vi "Start Record.vi"(8 "error in (no error)":errorcluster, 10 "tdms ref":refnum<k34>, 11 "DMM Engine":refnum<class "DMM Engine.lvclass">) -> (0 "error out":errorcluster, 3 "DMM Engine out":refnum<class "DMM Engine.lvclass">)   [LabVIEW 2025, in "DMM.lvlib" / "DMM Engine.lvclass"]
uses:
  DMM Engine.lvclass
  DMM Engine.lvclass/DMM Engine.ctl
  DMM configuration/DMM configuration.lvclass
  DMM Channel/DMM Channel.lvclass
  Users/Public/Documents/Sandia National Labs/TSS Plugin/Abstract.lvlibp/Channel configuration/Channel configuration.lvclass
  DMM Instrument/DMM Instrument.lvclass
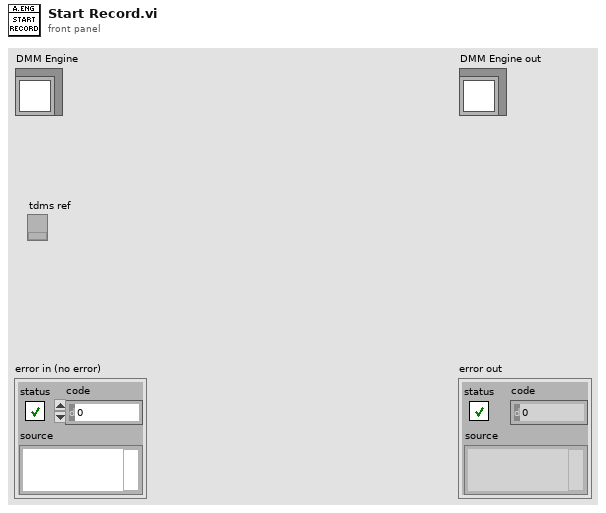
[diagram p1: front panel]
types:
  T1 = typedef "Abstract.lvlibp/Abstract Engine.lvclass/Engine Cluster.ctl" = cluster{"Initialized":bool, "IP Address":string, "Engine Type":string, "InstrumentMap":map{string, cluster{"Initialized":bool, "IP Address":string, "Instr Type":string, "Channels":cluster{"Enable":bool, "Alias":string}[]}}}
  T2 = typedef "Abstract.lvlibp/Instrument configuration.lvclass/Default Instrument.ctl" = cluster{"InstType":string, "Address":string, "SW Alias":string, "Description":string, "Enabled":bool}
  T3 = typedef "Abstract.lvlibp/Channel configuration.lvclass/Default Channel.ctl" = cluster{"SW Alias":string, "Enabled":bool, "Class":string, "Type":T4, "AI Parameter":cluster{"Upper limit":dbl, "Lower limit":dbl, "Unit":T4}}
  T4 = typedef "Abstract.lvlibp/Channel configuration.lvclass/Data Type.ctl" = string
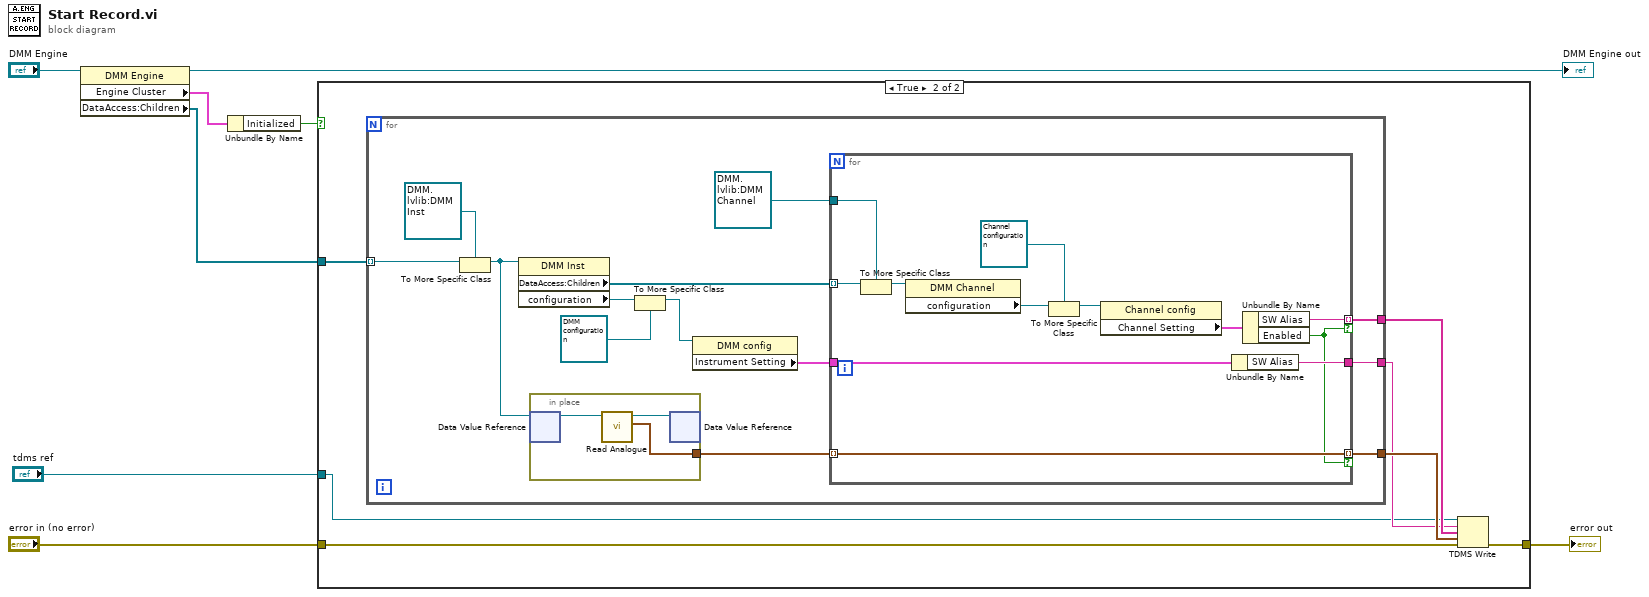
[diagram p0: block diagram]
diagram:
  n1 = property class="DMM Engine"(reference="DMM Engine") -> (reference out=→"DMM Engine out":refnum<class "DMM Engine.lvclass">, "Engine Cluster"=w5:T1, "DataAccess:Children"=w1:refnum<data-value>[])  [unwired: 1 in, 1 out]
  n2 = Unbundle By Name(w5) -> ("Initialized"=w8:bool)
  n3 = case shown="True" w8 {
    tunnel: "error in (no error)" -> [w9 w11]
    tunnel: [w9 w15] -> w6
    tunnel: "tdms ref" -> [_ w10]
    tunnel: w1 -> [_ w16]
    frame False {
    }
    frame True {
      n4 = for {
        tunnel: w16 -> [w26] mode=indexing
        tunnel: [w29] -> w14
        tunnel: [w28] -> w13
        tunnel: [w27] -> w12
        n5 = To More Specific Class(target class=refnum<data-value> refnum ("data value reference"), reference=w26) -> (specific class reference=w19:refnum<data-value>)  [unwired: 1 in, 1 out]
        n6 = property class="DMM Inst"(reference=w19) -> ("DataAccess:Children"=w20:refnum<data-value>[], "configuration"=w22:refnum<class "CEF_serializable configuration.lvclass">)  [unwired: 1 in, 2 out]
        n7 = in-place {
          in-place-border: [w30] -> w18
          n8 = in-place-dvr #1(w19) -> (w32:refnum<class "DMM Instrument.lvclass">)  [unwired: 1 out]
          n9 = call-dynamic "Read Analogue.vi"("Abstract DMM in"=w32) -> ("Waveforms"=w30:waveform(dbl)[], "Abstract DMM out"=w31:refnum<class "DMM Instrument.lvclass">)  [unwired: 8 in, 1 out]
          n10 = in-place-dvr #1(w31) -> ()  [unwired: 2 out]
        }
        n11 = To More Specific Class(target class=refnum<class "DMM configuration.lvclass"> refnum ("DMM.lvlib:DMM config"), reference=w22) -> (specific class reference=w24:refnum<class "DMM configuration.lvclass">)  [unwired: 1 in, 1 out]
        n12 = property class="DMM config"(reference=w24) -> ("Instrument Setting"=w21:T2)  [unwired: 1 in, 2 out]
        n13 = for {
          tunnel: w21 -> [w43]
          tunnel: w18 -> [w37] mode=indexing
          tunnel: [w37] -> w29 mode=indexing if=w35
          tunnel: [w38] -> w28 mode=indexing if=w35
          tunnel: [w36] -> w27
          tunnel: w20 -> [w34] mode=indexing
          tunnel: refnum<data-value> refnum ("data value reference") -> [w33]
          n14 = To More Specific Class(target class=w33, reference=w34) -> (specific class reference=w44:refnum<data-value>)  [unwired: 1 in, 1 out]
          n15 = property class="DMM Channel"(reference=w44) -> ("configuration"=w42:refnum<class "CEF_serializable configuration.lvclass">)  [unwired: 1 in, 2 out]
          n16 = To More Specific Class(target class=refnum<class "Channel configuration.lvclass"> refnum ("Abstract.lvlibp:Channel config"), reference=w42) -> (specific class reference=w40:refnum<class "Channel configuration.lvclass">)  [unwired: 1 in, 1 out]
          n17 = property class="Channel config"(reference=w40) -> ("Channel Setting"=w39:T3)  [unwired: 1 in, 2 out]
          n18 = Unbundle By Name(w43) -> ("SW Alias"=w36:string)
          n19 = Unbundle By Name(w39) -> ("SW Alias"=w38:string, "Enabled"=w35:bool)
        }
      }
      n20 = TDMS Write(0:w10, 5:w12, 7:w13, 9:w14, 11:w11) -> (15:w15:errorcluster)  [unwired: 1 in, 3 out]
    }
  }
  "error out" <- w6
